vi "MQTT Client - Subscribe.vi"(0 "MQTT Session":T4, 1 "No Local (v5)":bool, 2 "Retain As Published (v5)":bool, 3 "Retain Handling Options (v5)":T1(ring), 5 "Multiple Topics":cluster{"Topic Filter":string, "QoS":T3}[](array[cluster]), 7 "Single Topic Filter":string, 9 "Single Topic QoS":T3, 11 "error in (no error)":errorcluster, 12 "Subscribe Properties (v5)":T2[](array[typedef]) {"Property" items=[" Subscription Identifier           "=11, " User Property                     "=38]}) -> (4 "MQTT Session out":T4, 15 "error out":errorcluster)   [LabVIEW 2019, in "KoRE-MQTT.lvlib"]
doc: "<b>Description:</b> This VI subscribes to specific topics on an MQTT broker, enabling the client to receive messages published to those topics. It allows for different configurations for handling multiple topics and single topic subscriptions based on the user's requirements.\n\n<b>Input Terminals:</b>\n- <b>Retain Handling Options [3]</b>: Configuration setting for how retained messages are handled during subscriptions.\n- <b>Retain As Published (v5) [2]</b>: Boolean value indicating whether to retain messages according to the publish message's retain flag for MQTT v5 connections.\n- <b>No Local (v5) [1]</b>: Boolean value indicating that the server should not send a publish message back to this client if the message was originally sent from this client. Only applicable for MQTT v5 connections.\n- <b>MQTT Session [0]</b>: Reference to the MQTT session utilized for managing subscriptions.\n- <b>Multiple Topics [5]</b>: Array of topic filters and Quality of Service levels for subscribing to multiple topics.\n- <b>Single Topic Filter [7]</b>: Specific topic filter for subscribing to a single topic.\n- <b>Single Topic QoS [9]</b>: Quality of Service level for the single topic subscription.\n- <b>Properties (optional) [11]</b>: Array of Property and Value pairs for MQTT v5 connections used during subscription.\n\n<b>Output Terminals:</b>\n- <b>MQTT Session out [4]</b>: Reference to the active MQTT session.\n\n<b>Examples of MQTT Topic Filter strings:</b>\n\n<b>\"factory/+/temperature\"</b> \nSubscribes to all temperature readings from machines, enabling a manufacturing \nfacility to monitor temperatures across multiple machines, such as \n<b>factory/robot1/temperature</b>.\n\n<b>\"equipment/line1/#\"</b> \nSubscribes to all messages related to a specific production line. This allows \nfor comprehensive monitoring of all equipment statuses, including operational \nmetrics and alerts, like <b>equipment/line1/motor/status</b>.\n\n<b>\"sensors/+/status\"</b> \nSubscribes to status updates from various sensors. A centralized monitoring \nsystem can then track the operational health of sensors (e.g., vibration, \npressure) used in machinery.\n\n<b>\"machines/line1/power\"</b> \nSubscribes to power consumption messages for line1, allowing energy management \nsystems to evaluate and optimize power usage on specific production lines.\n\n<b>\"+/alarms\"</b> \nSubscribes to alarms from all machines. This function notifies operators about \ncritical conditions or malfunctions across all production units.\n\n<b>\"production/#\"</b> \nSubscribes to all messages related to production activities. This facilitates \ncomprehensive monitoring of production processes, including output data and \nefficiency metrics.\n\n<b>\"maintenance/+/schedule\"</b> \nSubscribes to maintenance schedules for all equipment, helping to facilitate \nproactive maintenance by providing schedules for regular checks and servicing \nacross all machines.\n\n\nCopyright (c) 2025 KoRElibs.com\nSPDX-License-Identifier: EUPL-1.2\n\nThis VI is licensed under the European Union Public License (EUPL) Version 1.2. You may use this VI unmodified in proprietary works. If you distribute a modified version of this file, the modified file must be released under the EUPL-1.2. Full license: https://joinup.ec.europa.eu/asset/eupl/eupl/1.2/"
uses:
  KoRE-MQTT.lvlib
  TypeDefs/MQTT QoS Level.ctl
  TypeDefs/MQTT Client Session.ctl
  TypeDefs/MQTT Property - SUBSCRIBE.ctl
  Private/TypeDefs/MQTT Packet - Type.ctl
  Private/MQTT Session - Get TCP Info.vi
  Private/MQTT Session - Reset Keep Alive Timer.vi
  Private/MQTT Data Stream - Write Packet.vi
  Private/MQTT Data - Encode Varint.vi
panel:
  out "DEBUG":string
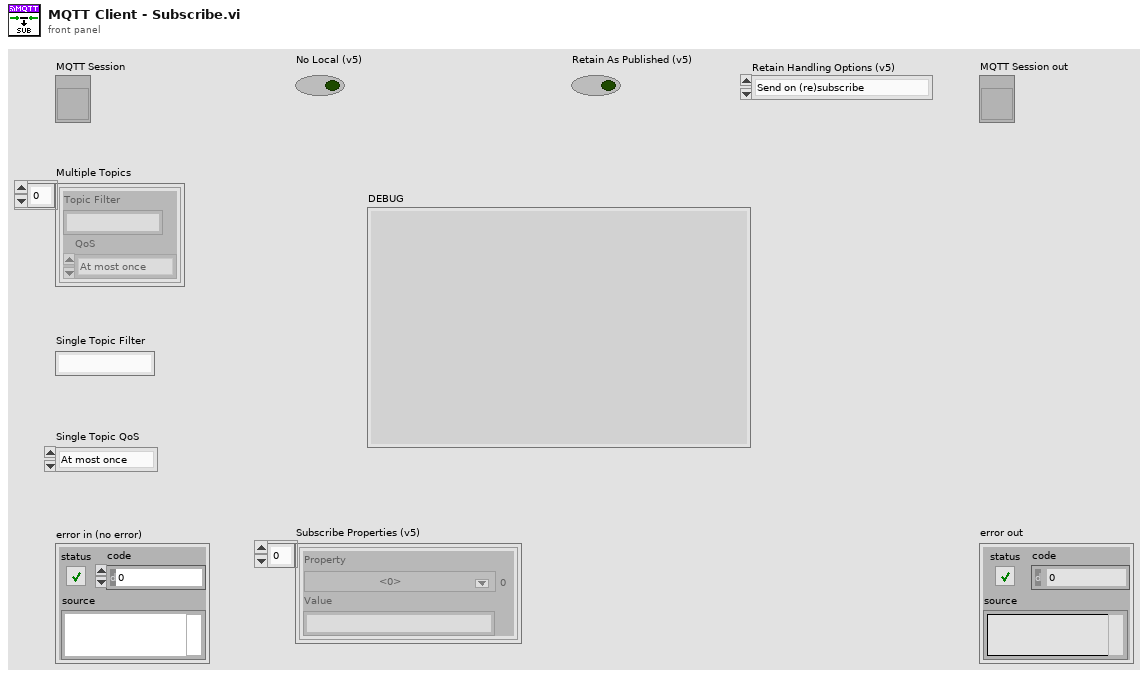
[diagram p1: front panel]
types:
  T1 = enum16{"Send on (re)subscribe", "Send on subscribe", "Do not send"}
  T2 = typedef "KoRE-MQTT.lvlib/MQTT Property - SUBSCRIBE.ctl" = cluster{"Property":u8, "Value":string}
  T3 = typedef "KoRE-MQTT.lvlib/MQTT QoS Level.ctl" = enum8{"At most once", "At least once", "Exactly once"}
  T4 = typedef "KoRE-MQTT.lvlib/MQTT Client Session.ctl" = refnum<vi>
  T5 = cluster{"Topic Filter":string, "Single Topic QoS":T3}[]
  T6 = typedef "KoRE-MQTT.lvlib/MQTT Packet - Type.ctl" = enum32{"Reserved", "CONNECT", "CONNACK", "PUBLISH", "PUBACK", "PUBREC", "PUBREL", "PUBCOMP", "SUBSCRIBE", "SUBACK", "UNSUBSCRIBE", "UNSUBACK", "PINGREQ", "PINGRESP", "DISCONNECT", "AUTH"}
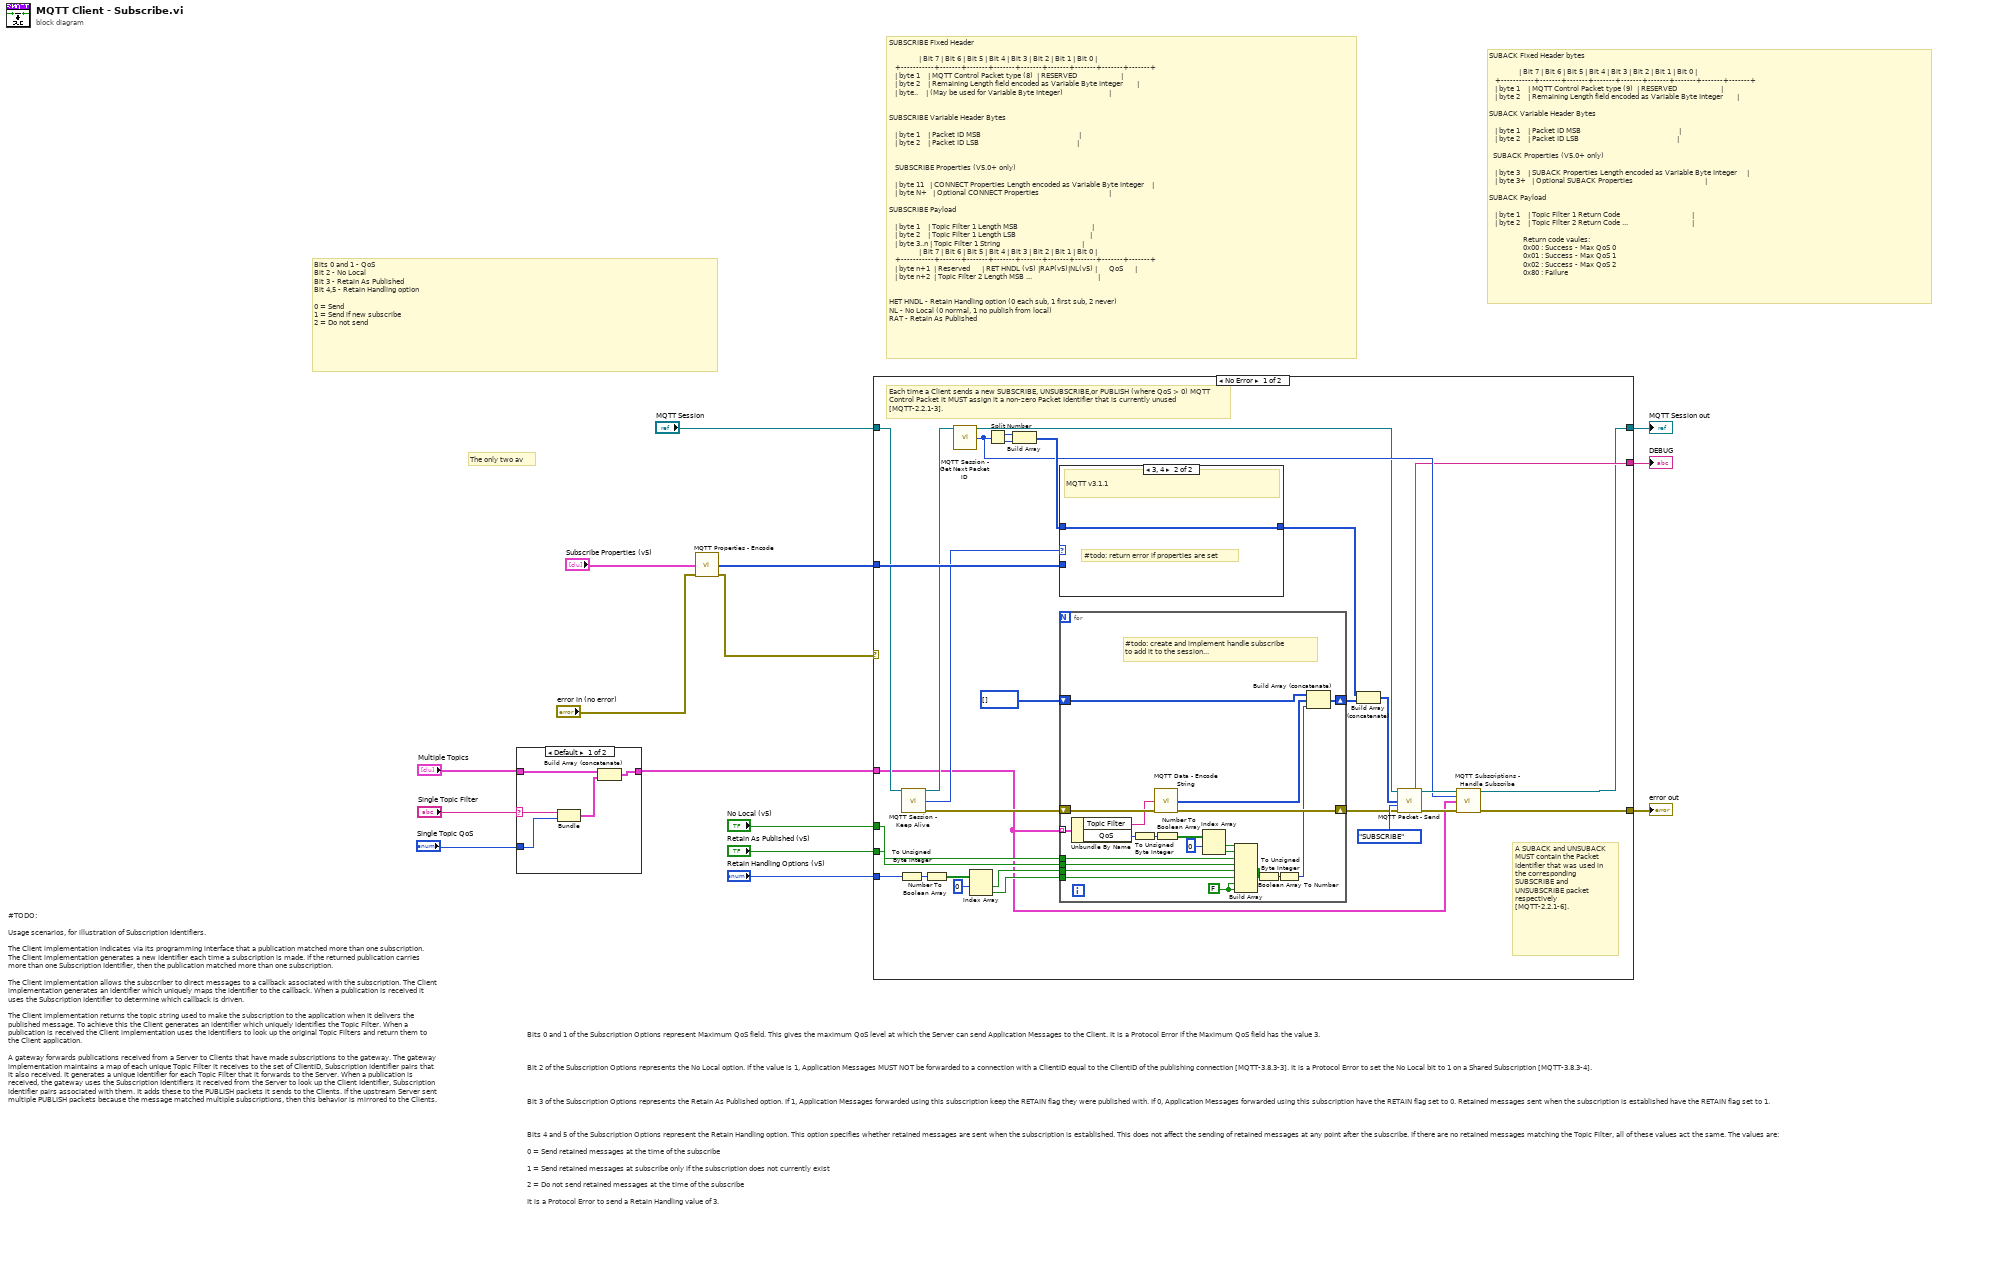
[diagram p0: block diagram]
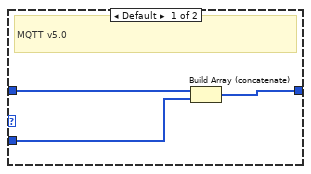
[diagram p2: hidden frame]
diagram:
  # "SUBSCRIBE Fixed Header\n\n               | Bit 7 | Bit 6 | Bit 5 | Bit 4 | Bit 3 | Bit 2 | Bit 1 | Bit 0 |\n   +-----------+-------+-------+-------+-------+-------+-------+-------+-------+\n   | byte 1    | MQTT Control Packet type (8)  | RESERVED                      |\n   | byte 2    | Remaining Length field encoded as Variable Byte Integer       |\n   | byte..    | (May be used for Variable Byte Integer)                       | \n\n\nSUBSCRIBE Variable Header Bytes\n\n   | byte 1    | Packet ID MSB                                                 |  \n   | byte 2    | Packet ID LSB                                                 |\n\n\n   SUBSCRIBE Properties (V5.0+ only)\n\n   | byte 11   | CONNECT Properties Length encoded as Variable Byte Integer    |\n   | byte N+   | Optional CONNECT Properties                                   |\n\nSUBSCRIBE Payload \n\n   | byte 1    | Topic Filter 1 Length MSB                                     |\n   | byte 2    | Topic Filter 1 Length LSB                                     |\n   | byte 3..n | Topic Filter 1 String                                         |\n               | Bit 7 | Bit 6 | Bit 5 | Bit 4 | Bit 3 | Bit 2 | Bit 1 | Bit 0 |\n   +-----------+-------+-------+-------+-------+-------+-------+-------+-------+\n   | byte n+1  | Reserved      | RET HNDL (v5) |RAP(v5)|NL(v5) |      QoS      |\n   | byte n+2  | Topic Filter 2 Length MSB ...                                 |\n \n\nHET HNDL - Retain Handling option (0 each sub, 1 first sub, 2 never)\nNL - No Local (0 normal, 1 no publish from local)\nRAT - Retain As Published"
  # "Bits 0 and 1 - QoS\nBit 2 - No Local\nBit 3 - Retain As Published\nBit 4,5 - Retain Handling option\n\n0 = Send\n1 = Send if new subscribe\n2 = Do not send"
  # "Bits 0 and 1 of the Subscription Options represent Maximum QoS field. This gives the maximum QoS level at which the Server can send Application Messages to the Client. It is a Protocol Error if the Maximum QoS field has the value 3.\n\n \n\nBit 2 of the Subscription Options represents the No Local option. If the value is 1, Application Messages MUST NOT be forwarded to a connection with a ClientID equal to the ClientID of the publishing connection [MQTT-3.8.3-3]. It is a Protocol Error to set the No Local bit to 1 on a Shared Subscription [MQTT-3.8.3-4].\n\n \n\nBit 3 of the Subscription Options represents the Retain As Published option. If 1, Application Messages forwarded using this subscription keep the RETAIN flag they were published with. If 0, Application Messages forwarded using this subscription have the RETAIN flag set to 0. Retained messages sent when the subscription is established have the RETAIN flag set to 1.\n\n \n\nBits 4 and 5 of the Subscription Options represent the Retain Handling option. This option specifies whether retained messages are sent when the subscription is established. This does not affect the sending of retained messages at any point after the subscribe. If there are no retained messages matching the Topic Filter, all of these values act the same. The values are:\n\n0 = Send retained messages at the time of the subscribe\n\n1 = Send retained messages at subscribe only if the subscription does not currently exist\n\n2 = Do not send retained messages at the time of the subscribe\n\nIt is a Protocol Error to send a Retain Handling value of 3."
  # "#TODO: \n\nUsage scenarios, for illustration of Subscription Identifiers.\n\nThe Client implementation indicates via its programming interface that a publication matched more than one subscription. The Client implementation generates a new identifier each time a subscription is made. If the returned publication carries more than one Subscription Identifier, then the publication matched more than one subscription.\n\nThe Client implementation allows the subscriber to direct messages to a callback associated with the subscription. The Client implementation generates an identifier which uniquely maps the identifier to the callback. When a publication is received it uses the Subscription Identifier to determine which callback is driven.\n\nThe Client implementation returns the topic string used to make the subscription to the application when it delivers the published message. To achieve this the Client generates an identifier which uniquely identifies the Topic Filter. When a publication is received the Client implementation uses the identifiers to look up the original Topic Filters and return them to the Client application.\n\nA gateway forwards publications received from a Server to Clients that have made subscriptions to the gateway. The gateway implementation maintains a map of each unique Topic Filter it receives to the set of ClientID, Subscription Identifier pairs that it also received. It generates a unique identifier for each Topic Filter that it forwards to the Server. When a publication is received, the gateway uses the Subscription Identifiers it received from the Server to look up the Client Identifier, Subscription Identifier pairs associated with them. It adds these to the PUBLISH packets it sends to the Clients. If the upstream Server sent multiple PUBLISH packets because the message matched multiple subscriptions, then this behavior is mirrored to the Clients."
  # "The only two av"
  # "SUBACK Fixed Header bytes\n\n               | Bit 7 | Bit 6 | Bit 5 | Bit 4 | Bit 3 | Bit 2 | Bit 1 | Bit 0 |\n   +-----------+-------+-------+-------+-------+-------+-------+-------+-------+\n   | byte 1    | MQTT Control Packet type (9)  | RESERVED                      |\n   | byte 2    | Remaining Length field encoded as Variable Byte Integer       |\n\nSUBACK Variable Header Bytes\n\n   | byte 1    | Packet ID MSB                                                 |  \n   | byte 2    | Packet ID LSB                                                 |\n\n  SUBACK Properties (V5.0+ only)\n\n   | byte 3    | SUBACK Properties Length encoded as Variable Byte Integer     |\n   | byte 3+   | Optional SUBACK Properties                                    |\n\nSUBACK Payload \n\n   | byte 1    | Topic Filter 1 Return Code                                    |\n   | byte 2    | Topic Filter 2 Return Code ...                                |\n\n                 Return code vaules: \n                 0x00 : Success - Max QoS 0\n                 0x01 : Success - Max QoS 1\n                 0x02 : Success - Max QoS 2\n                 0x80 : Failure"
  n1 = case shown="Default" "Single Topic Filter" {
    selector: "Single Topic Filter" -> [w19 _]
    tunnel: "Multiple Topics" -> [w20 w21]
    tunnel: [w16 w21] -> w10
    tunnel: "Single Topic QoS" -> [w17 _]
    frame Default {
      n2 = Bundle(w19, "Single Topic QoS"=w17) -> (w18:cluster{string, "Single Topic QoS":T3})  [unwired: 1 in]
      n3 = Build Array (concatenate)(w20, w18) -> (w16:T5)
    }
    frame "" {
    }
  }
  n4 = call "MQTT Properties - Encode.vi"("MQTT Properties"="Subscribe Properties (v5)", "error in (no error)"="error in (no error)") -> ("Encoded MQTT Properties"=w7:u8[], "error out"=w5:errorcluster)  [unwired: 12 in]
  n5 = case shown="No Error" w5 {
    selector: w5 -> [_ w78]
    tunnel: [w26 w78] -> w15
    tunnel: "MQTT Session" -> [w45 w77]
    tunnel: w10 -> [w32 _]
    tunnel: [w25 w77] -> w13
    tunnel: w7 -> [w47 _]
    tunnel: "No Local (v5)" -> [w40 _]
    tunnel: "Retain Handling Options (v5)" -> [w41 _]
    tunnel: "Retain As Published (v5)" -> [w39 _]
    tunnel: [w29 _] -> w1
    frame No Error {
      # "A SUBACK and UNSUBACK MUST contain the Packet Identifier that was used in the corresponding SUBSCRIBE and UNSUBSCRIBE packet respectively [MQTT-2.2.1-6]."
      # "Each time a Client sends a new SUBSCRIBE, UNSUBSCRIBE,or PUBLISH (where QoS > 0) MQTT Control Packet it MUST assign it a non-zero Packet Identifier that is currently unused [MQTT-2.2.1-3]."
      n6 = To Unsigned Byte Integer(number=w41) -> (unsigned 8bit integer=w42:u8)
      n7 = call "MQTT Session - Keep Alive.vi"("mqtt ref in"=w45) -> ("mqtt ref out"=w46:T4, "Version"=w44:u8, "error out"=w43:errorcluster)  [unwired: 12 in]
      n8 = Number To Boolean Array(number=w42) -> (Boolean array=w37:bool[])
      n9 = call "MQTT Session - Get Next Packet ID.vi"("MQTT_Q In in"=w46) -> ("MQTT_Q In out"=w28:T4, "PacketID"=w30:u16)  [unwired: 13 in]
      n10 = Index Array(array=w37, index #1=0 ("index")) -> (element #1=w38:bool, element #2=w36:bool)  [unwired: 1 in]
      n11 = Split Number(x=w30) -> (hi(x)=w50:u8, lo(x)=w51:u8)
      n12 = Build Array(w50, w51) -> (w31:u8[])
      n13 = for {
        shift-right: [w75] -> w27
        shift-left: w43 -> [w76]
        shift-right: [w74] -> w24
        shift-left: u8[] [] -> [w59]
        tunnel: w32 -> [w73] mode=indexing
        tunnel: w40 -> [w65]
        tunnel: w39 -> [w64]
        tunnel: w38 -> [w62]
        tunnel: w36 -> [w61]
        w63 = FALSE
        # "#todo: create and implement handle subscribe \nto add it to the session..."
        n14 = Unbundle By Name(w73) -> ("Topic Filter"=w56:string, "QoS"=w72:T3)
        n15 = To Unsigned Byte Integer(number=w72) -> (unsigned 8bit integer=w71:u8)
        n16 = call "MQTT Data - Encode String.vi"("String in"=w56, "error in (no error)"=w76) -> ("Bytes out"=w58:u8[], "error out"=w75:errorcluster)  [unwired: 12 in]
        n17 = Number To Boolean Array(number=w71) -> (Boolean array=w68:bool[])
        n18 = Index Array(array=w68, index #1=0 ("index")) -> (element #1=w67:bool, element #2=w66:bool)  [unwired: 1 in]
        n19 = Build Array(w67, w66, w65, w64, w62, w61, w63, w63) -> (w70:bool[])
        n20 = Boolean Array To Number(Boolean array=w70) -> (number=w69:u32)
        n21 = To Unsigned Byte Integer(number=w69) -> (unsigned 8bit integer=w57:u8)
        n22 = Build Array (concatenate)(w59, w58, w57) -> (w74:u8[])
      }
      n23 = case shown="3, 4" w44 {
        tunnel: w31 -> [w54 w55]
        tunnel: [w53 w55] -> w23
        tunnel: w47 -> [w52 _]
        frame Default {
          # "MQTT v5.0"
          n24 = Build Array (concatenate)(w54, w52) -> (w53:u8[])
        }
        frame 3, 4 {
          # "#todo: return error if properties are set"
          # "MQTT v3.1.1"
        }
      }
      n25 = Build Array (concatenate)(w23, w24) -> (w22:u8[])
      n26 = call "MQTT Packet - Send.vi"("mqtt ref in"=w28, "packet data"=w22, "MessageType"=MQTT_Packet_-_Type."SUBSCRIBE", "error in (no error)"=w27) -> ("Debug"=w29:string, "mqtt ref out"=w34:T4, "error out"=w33:errorcluster)  [unwired: 9 in]
      n27 = call "MQTT Subscriptions - Handle Subscribe.vi"("MQTT ref in"=w34, "Packet ID"=w30, "Subscriptions"=w32, "error in"=w33) -> ("MQTT ref out"=w25:T4, "error out"=w26:errorcluster)  [unwired: 10 in]
    }
    frame Error {
    }
  }
  "error out" <- w15
  "MQTT Session out" <- w13
  "DEBUG" <- w1
